vi "test.vi"() -> ()   [LabVIEW 2020]
uses:
  <vilib>/drjdpowell/SQLite Library/SQL Statement/SQLITE Datatype.ctl
  <vilib>/drjdpowell/SQLite Library/SQL Statement/SQL Statement.lvclass/SQL Statement.ctl
  <vilib>/drjdpowell/SQLite Library/SQL Connection/Open (string).vi
  <vilib>/drjdpowell/SQLite Library/SQL Statement/Column Type_decl.vi
  <vilib>/drjdpowell/SQLite Library/SQL Statement/Column Type.vi
  <vilib>/drjdpowell/SQLite Library/SQL Statement/Next Bind (name).vi
  <vilib>/drjdpowell/SQLite Library/SQL Statement/Get Column Names.vi
  <vilib>/drjdpowell/SQLite Library/SQL Statement/Next Bind.vi
  <vilib>/drjdpowell/SQLite Library/SQL Statement/Get Column Count.vi
  <vilib>/drjdpowell/SQLite Library/SQL Statement/Write Next Column.vi
  <vilib>/drjdpowell/SQLite Library/SQL Statement/Get Column Name.vi
  <vilib>/drjdpowell/SQLite Library/SQL Connection/Execute SQL (No results).vi
  <vilib>/drjdpowell/SQLite Library/SQL Statement/Bind Parameters.vi
  <vilib>/drjdpowell/SQLite Library/SQL Statement/Error Message.vi
  <vilib>/drjdpowell/SQLite Library/SQL Connection/Execute SQL.vi
  <vilib>/drjdpowell/SQLite Library/SQL Statement/Column Variant.vi
  <vilib>/drjdpowell/SQLite Library/SQL Connection/Connection.lvclass
  <vilib>/drjdpowell/SQLite Library/SQLite.lvlib
  <vilib>/drjdpowell/SQLite Library/SQL Statement/SQL Statement.lvclass
panel:
  out "Array 4":string[][](array[string])
  out "Array 3":T1[][](array[typedef])
  out "Array 2":variant[][](array[variant])
  out "Array":variant[](array[variant])
  out "Row returned":bool
  out "Result Set":string[][](array[string])
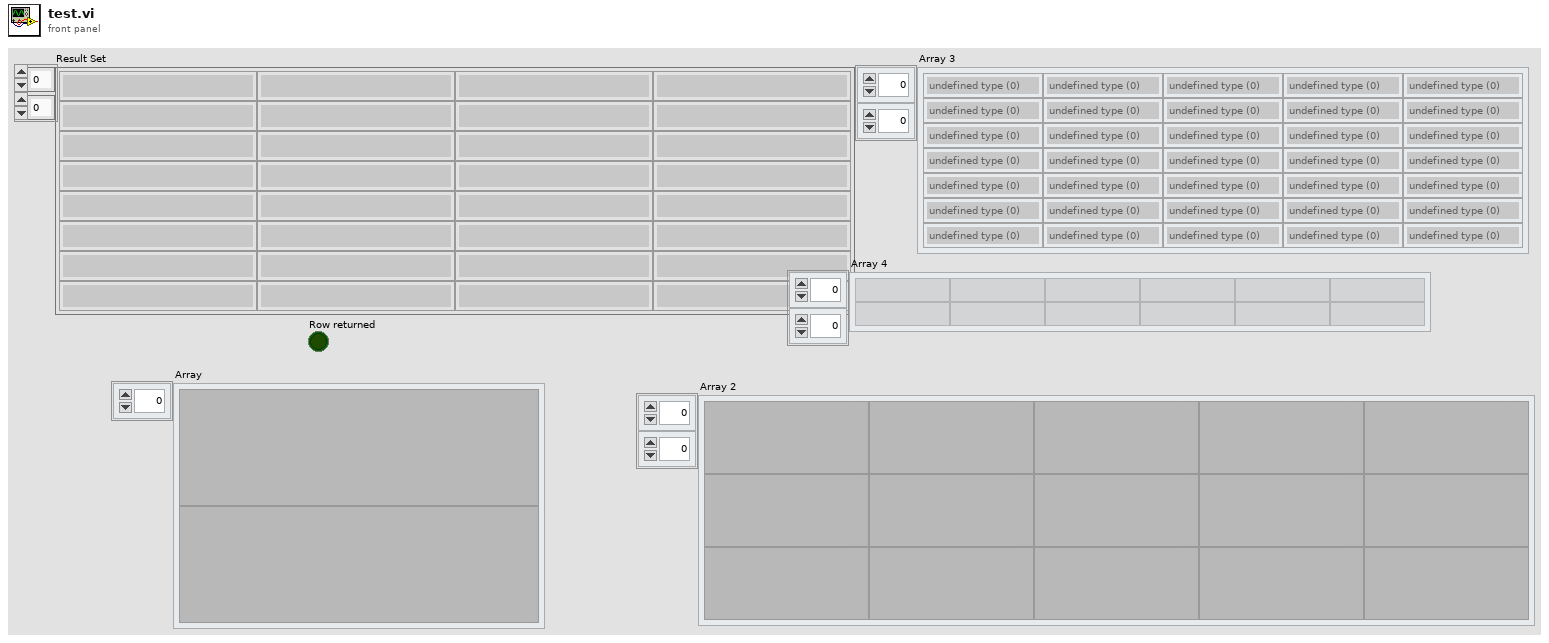
[diagram p1: front panel]
types:
  T1 = typedef "SQLite.lvlib/SQL Statement.lvclass/SQLITE Datatype.ctl" = enum32{"undefined type (0)", "SQLITE_INTEGER", "SQLITE_FLOAT", "SQLITE3_TEXT", "SQLITE_BLOB", "SQLITE_NULL", "undefined type"}
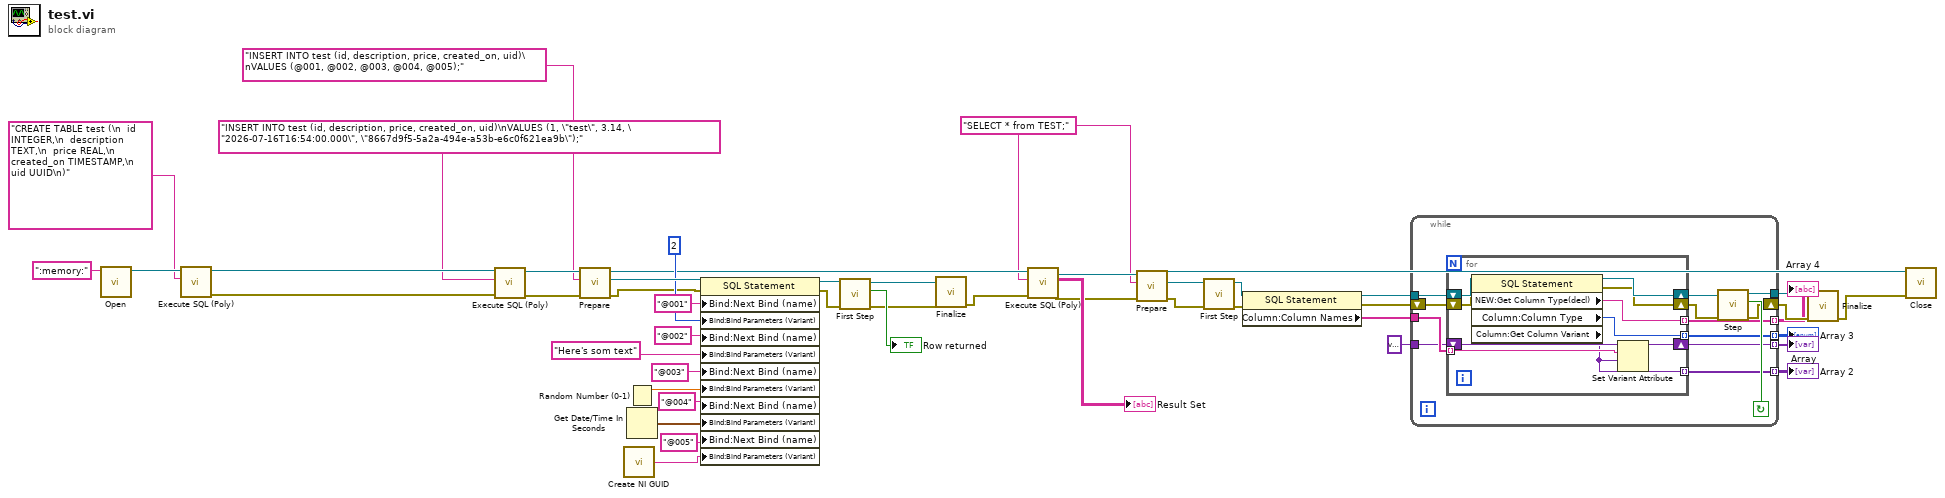
[diagram p0: block diagram]
diagram:
  w19 = "SELECT * from TEST;" ("SQL")
  n1 = call-poly <vilib>:"Open.vi"("db file"=":memory:") -> ("SQLite Connection"=w47:refnum<class "Connection.lvclass">)  [unwired: 9 in, 1 out]
  n2 = call-poly <vilib>:"Execute SQL (Poly).vi"("SQL"="CREATE TABLE test (\n  id INTEGER,\n  description TEXT,\n  price REAL,\n  created_on TIMESTAMP,\n  uid UUID\n)", "SQLite Connection in"=w47) -> ("error out"=w44:errorcluster, "SQLite Connection"=w45:refnum<class "Connection.lvclass">)  [unwired: 8 in]
  n3 = call-poly <vilib>:"Execute SQL (Poly).vi"("error in (no error)"=w44, "SQL"="INSERT INTO test (id, description, price, created_on, uid)\nVALUES (1, \"test\", 3.14, \"2026-07-16T16:54:00.000\", \"8667d9f5-5a2a-494e-a53b-e6c0f621ea9b\");", "SQLite Connection in"=w45) -> ("error out"=w40:errorcluster, "SQLite Connection"=w41:refnum<class "Connection.lvclass">)  [unwired: 7 in]
  n4 = call <vilib>:"Prepare.vi"("error in (no error)"=w40, "SQL"="INSERT INTO test (id, description, price, created_on, uid)\nVALUES (@001, @002, @003, @004, @005);", "SQLite Connection in"=w41) -> ("error out"=w24:errorcluster, "SQL Statement"=w38:refnum<class "SQL Statement.lvclass">, "SQLite Connection"=w25:refnum<class "Connection.lvclass">)  [unwired: 4 in, 2 out]
  n5 = call <vilib>:"Create NI GUID.vi"() -> ("NI GUID"=w2:string)
  n6 = Random Number (0-1)() -> (number: 0 to 1=w32:dbl)
  n7 = Get Date/Time In Seconds() -> (seconds since 1Jan1904=w23:timestamp)
  n8 = property class="SQL Statement"(reference=w38, error in=w24, "Bind:Next Bind (name)"="@001" ("Next Bind (name)"), "Bind:Bind Parameters (Variant)"=i64 2 ("Bind:Integer"), "Bind:Next Bind (name)"="@002" ("Next Bind (name)"), "Bind:Bind Parameters (Variant)"="Here's som text" ("Next Bind (name)"), "Bind:Next Bind (name)"="@003" ("Next Bind (name)"), "Bind:Bind Parameters (Variant)"=w32, "Bind:Next Bind (name)"="@004" ("Next Bind (name)"), "Bind:Bind Parameters (Variant)"=w23, "Bind:Next Bind (name)"="@005" ("Next Bind (name)"), "Bind:Bind Parameters (Variant)"=w2) -> (reference out=w30:refnum<class "SQL Statement.lvclass">, error out=w31:errorcluster)
  n9 = call <vilib>:"First Step.vi"("error in (no error)"=w31, "SQL Statement in"=w30) -> ("error out"=w27:errorcluster, "Row returned"=→"Row returned":bool, "SQL Statement"=w28:refnum<class "SQL Statement.lvclass">)  [unwired: 7 in]
  n10 = call <vilib>:"Finalize.vi"("error in (no error)"=w27, "SQL Statement in"=w28) -> ("error out"=w26:errorcluster)  [unwired: 9 in]
  n11 = call-poly <vilib>:"Execute SQL (Poly).vi"("error in (no error)"=w26, "SQL"=w19, "SQLite Connection in"=w25) -> ("error out"=w20:errorcluster, "Result Set"=→"Result Set":string[][], "SQLite Connection"=w21:refnum<class "Connection.lvclass">)  [unwired: 5 in, 1 out]
  n12 = call <vilib>:"Prepare.vi"("error in (no error)"=w20, "SQL"=w19, "SQLite Connection in"=w21) -> ("error out"=w17:errorcluster, "SQL Statement"=w18:refnum<class "SQL Statement.lvclass">, "SQLite Connection"=w6:refnum<class "Connection.lvclass">)  [unwired: 4 in, 2 out]
  n13 = call <vilib>:"First Step.vi"("error in (no error)"=w17, "SQL Statement in"=w18) -> ("error out"=w15:errorcluster, "SQL Statement"=w16:refnum<class "SQL Statement.lvclass">)  [unwired: 7 in, 1 out]
  n14 = property class="SQL Statement"(reference=w16, error in=w15) -> (reference out=w14:refnum<class "SQL Statement.lvclass">, error out=w13:errorcluster, "Column:Column Names"=w12:string[])
  n15 = while {
    tunnel: w14 -> [w61]
    tunnel: [w59] -> w9
    shift-right: [w55] -> w8
    shift-left: w13 -> [w57]
    tunnel: w12 -> [w54]
    tunnel: variant -> [w53]
    tunnel: [w52] -> w10 mode=indexing
    tunnel: [w51] -> w4 mode=indexing
    tunnel: [w50] -> w5 mode=indexing
    tunnel: [w49] -> w1 mode=indexing
    stop <- w58 continue-if-true
    n16 = for {
      shift-right: [w70] -> w60
      shift-left: w61 -> [w71]
      shift-right: [w68] -> w56
      shift-left: w57 -> [w69]
      tunnel: w54 -> [w67] mode=indexing
      shift-right: [w66] -> w52
      shift-left: w53 -> [w65]
      tunnel: [w63] -> w51 mode=indexing
      tunnel: [w64] -> w50 mode=indexing
      tunnel: [w62] -> w49 mode=indexing
      n17 = property class="SQL Statement"(reference=w71, error in=w69) -> (reference out=w70:refnum<class "SQL Statement.lvclass">, error out=w68:errorcluster, "NEW:Get Column Type(decl)"=w62:string, "Column:Column Type"=w63:T1, "Column:Get Column Variant"=w64:variant)
      n18 = Set Variant Attribute(Variant=w65, name=w67, value=w64) -> (Variant out=w66:variant)  [unwired: 1 in, 2 out]
    }
    n19 = call <vilib>:"Step.vi"("error in (no error)"=w56, "SQL Statement in"=w60) -> ("error out"=w55:errorcluster, "Row returned"=w58:bool, "SQL Statement"=w59:refnum<class "SQL Statement.lvclass">)  [unwired: 7 in]
  }
  "Array" <- w10
  "Array 2" <- w5
  "Array 3" <- w4
  "Array 4" <- w1
  n20 = call <vilib>:"Finalize.vi"("error in (no error)"=w8, "SQL Statement in"=w9) -> ("error out"=w7:errorcluster)  [unwired: 9 in]
  n21 = call-dynamic "Close.vi"("error in (no error)"=w7, "SQLite Connection in"=w6) -> ()  [unwired: 9 in, 1 out]
